vi "query Center Frequency.vi"(8 "error in (no error)":errorcluster, 11 "Keysight 9020A in":refnum<class "Keysight 9020A.lvclass">) -> (0 "error out":errorcluster, 2 "Center Frequency (Hz)":dbl, 3 "Keysight 9020A out":refnum<class "Keysight 9020A.lvclass">)   [LabVIEW 2023, in "Spectrum Analyzer.lvlib" / "Keysight 9020A.lvclass"]
uses:
  Keysight 9020A.lvclass
  Keysight 9020A.lvclass/Keysight 9020A.ctl
  Spectrum Analyzer.lvlib
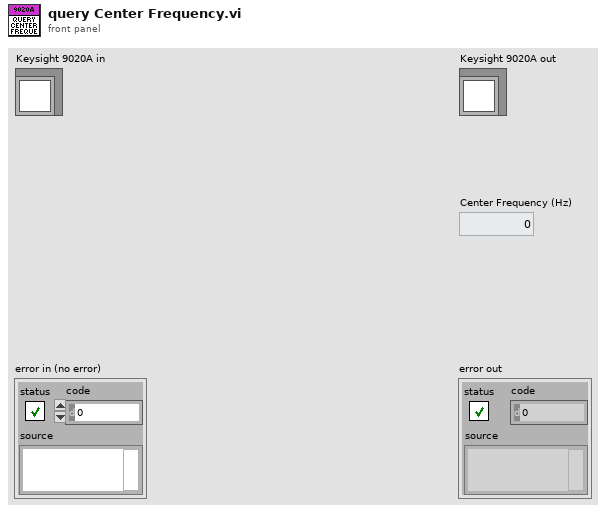
[diagram p1: front panel]
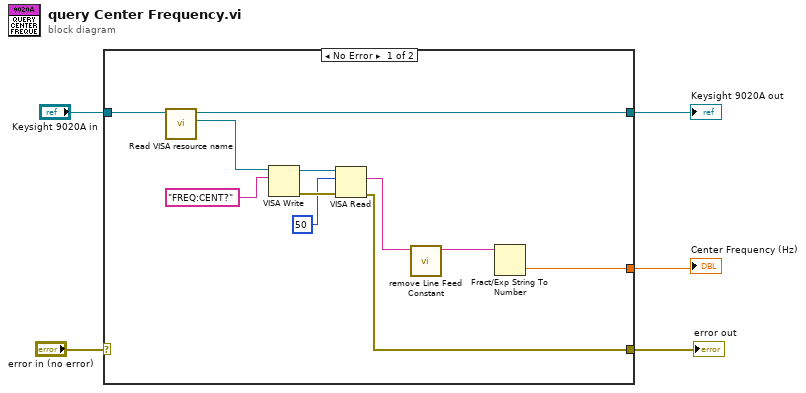
[diagram p0: block diagram]
diagram:
  n1 = case shown="No Error" "error in (no error)" {
    selector: "error in (no error)" -> [_ w17]
    tunnel: "Keysight 9020A in" -> [w16 w18]
    tunnel: [w15 w18] -> w4
    tunnel: [w9 w17] -> w2
    tunnel: [w6 _] -> w1
    frame No Error {
      n2 = call "Read VISA resource name.vi"("Keysight 9020A in"=w16) -> ("VISA resource name"=w7:refnum<visa-resource-name>, "Keysight 9020A out"=w15:refnum<class "Keysight 9020A.lvclass">)  [unwired: 8 in, 1 out]
      n3 = VISA Write(VISA resource name=w7, write buffer="FREQ:CENT?") -> (VISA resource name out=w13:refnum<visa-resource-name>, error out=w12:errorcluster)  [unwired: 1 in, 1 out]
      n4 = VISA Read(VISA resource name=w13, byte count=u32 50, error in (no error)=w12) -> (read buffer=w10:string, error out=w9:errorcluster)  [unwired: 2 out]
      n5 = call "remove Line Feed Constant.vi"("Input String"=w10) -> ("Line Feed Removed String"=w8:string)  [unwired: 10 in]
      n6 = Fract/Exp String To Number(string=w8) -> (number=w6:dbl)  [unwired: 3 in, 1 out]
    }
    frame Error {
    }
  }
  "error out" <- w2
  "Keysight 9020A out" <- w4
  "Center Frequency (Hz)" <- w1
